vi "W06_Judge.vi"() -> ()   [LabVIEW 2018]
doc: "Use this template to build a VI to use as a subVI."
panel:
  out "error out":errorcluster
  in  "CSV file":path
  out "CSV line":string
  out "first fail":string
  out "result":string
  out "PASS":bool
  in  "measurements T01..T05":dbl[](array[numeric])
  out "serial OK":bool
  in  "serial number":string
  # "Measure_All.vi is replaced by the array control: type the 5 measurements T01..T05."
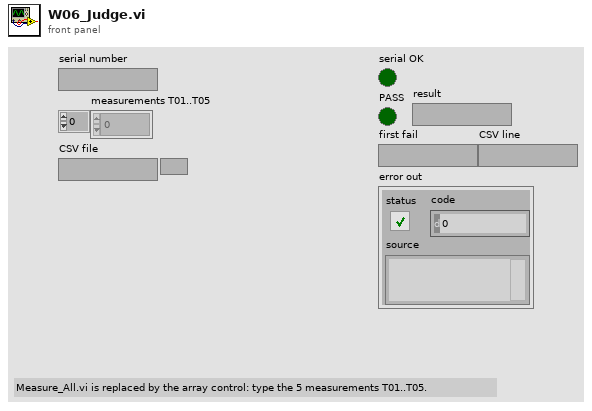
[diagram p1: front panel]
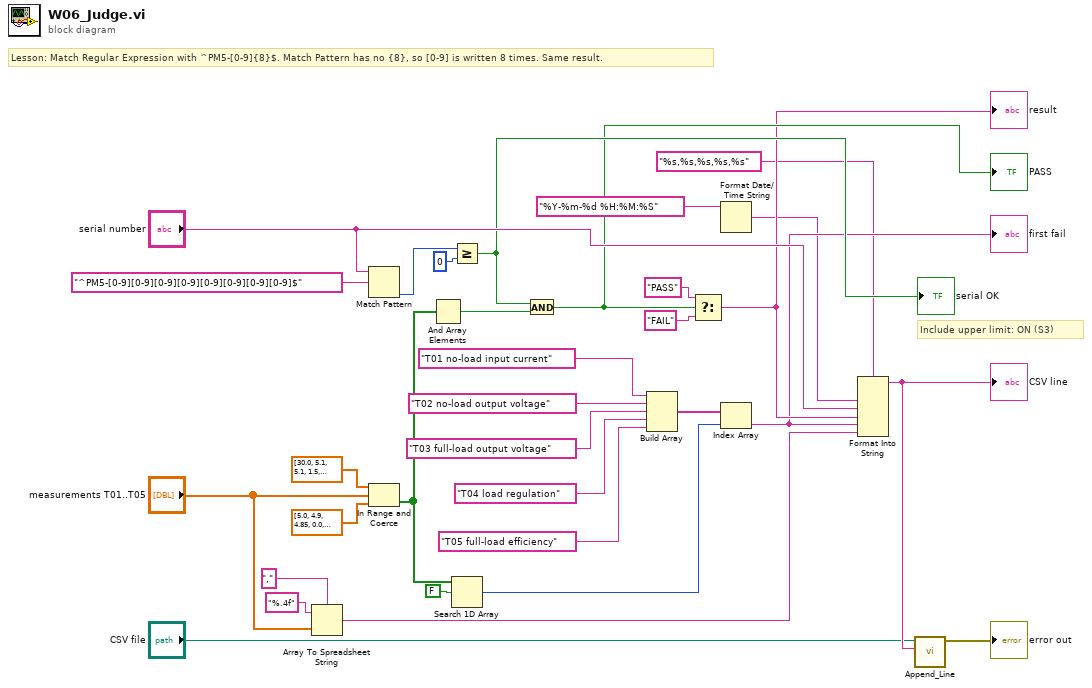
[diagram p0: block diagram]
diagram:
  # "Include upper limit: ON (S3)"
  # "Lesson: Match Regular Expression with ^PM5-[0-9]{8}$. Match Pattern has no {8}, so [0-9] is written 8 times. Same result."
  n1 = Array To Spreadsheet String(delimiter (Tab)=",", array="measurements T01..T05", 3:"%.4f") -> (spreadsheet string=w4:string)
  n2 = Match Pattern(string="serial number", regular expression="^PM5-[0-9][0-9][0-9][0-9][0-9][0-9][0-9][0-9]$") -> (offset past match=w30:i32)  [unwired: 1 in, 3 out]
  n3 = In Range and Coerce(upper limit=dbl[] [30.0, 5.1, 5.1, 1.5, 100.0], x="measurements T01..T05", lower limit=dbl[] [5.0, 4.9, 4.85, 0.0, 85.0]) -> (In Range?=w24:bool[])  [unwired: 1 out]
  n4 = And Array Elements(Boolean array=w24) -> (logical AND=w23:bool)
  n5 = Greater Or Equal?(x=w30, y=0) -> (x >= y?=w28:bool)
  "serial OK" <- w28
  n6 = Search 1D Array(1D array=w24, element=FALSE) -> (index of element=w11:i32)  [unwired: 1 in]
  n7 = And(x=w28, y=w23) -> (x .and. y?=w22:bool)
  "PASS" <- w22
  n8 = Build Array("T01 no-load input current", "T02 no-load output voltage", "T03 full-load output voltage", "T04 load regulation", "T05 full-load efficiency") -> (w12:string[])
  n9 = Select(t="PASS", s=w22, f="FAIL") -> (s? t:f=w19:string)
  "result" <- w19
  n10 = Format Date/Time String(time format string (%c)="%Y-%m-%d %H:%M:%S") -> (date/time string=w5:string)  [unwired: 2 in]
  n11 = Index Array(array=w12, index=w11) -> (element=w10:string)
  "first fail" <- w10
  n12 = Format Into String(format string="%s,%s,%s,%s,%s", w5, "serial number", w19, w10, w4) -> (resulting string=w3:string)  [unwired: 2 in, 1 out]
  "CSV line" <- w3
  n13 = call "Append_Line.vi"("text"=w3, "file path"="CSV file") -> ("error out"=→"error out":errorcluster)  [unwired: 9 in]
